vi "CfgManager Main Test Suite.vi"() -> ()   [LabVIEW 2013]
uses:
  source/Cache/ConfigManager.Cache.lvclass
  <vilib>/addons/_JKI Toolkits/Caraya/classes/Assert/Assert Equal Value and Type_Variant.vi
  <vilib>/addons/_JKI Toolkits/Caraya/classes/Assert/Assert Almost Equal_Float.vi
  source/Manager/Write.vi
  source/Manager/ConfigManager.lvclass
  <vilib>/addons/_JKI Toolkits/Caraya/classes/Test/Test.lvclass
  <vilib>/addons/_JKI Toolkits/Caraya/classes/Assert/Assert.lvclass
panel:
  out "error out":errorcluster
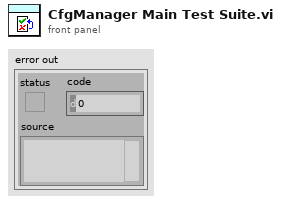
[diagram p1: front panel]
types:
  T1 = cluster{"P":dbl, "I":dbl, "D":dbl, "Type":enum16{"Manual", "Automatic"}}
  T2 = cluster{"P":dbl, "Type":enum16{"Manual", "Automatic"}}
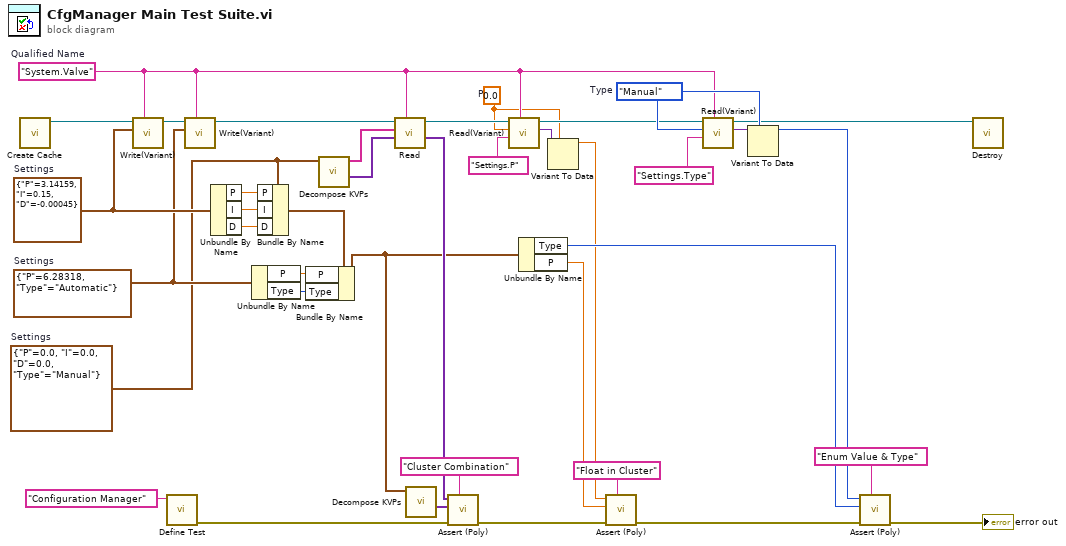
[diagram p0: block diagram]
diagram:
  w13 = 0.0  # P
  w1 = T1 {"P"=0.0, "I"=0.0, "D"=0.0, "Type"=enum."Manual"}  # Settings
  w32 = enum16{"Manual", "Automatic"}."Manual"  # Type
  w6 = T2 {"P"=6.28318, "Type"=enum."Automatic"}  # Settings
  w11 = cluster{"P":dbl, "I":dbl, "D":dbl} {"P"=3.14159, "I"=0.15, "D"=-0.00045}  # Settings
  w26 = "System.Valve"  # Qualified Name
  n1 = call "Create Cache.vi"() -> ("ConfigManager.Cache"=w39:refnum<class "ConfigManager.Cache.lvclass">)  [unwired: 11 in]
  n2 = call "Write(Variant).vi"("Qualified Name"=w26, "value"=w11, "ConfigManager in"=w39) -> ("ConfigManager out"=w35:refnum<class "ConfigManager.Cache.lvclass">)  [unwired: 6 in, 2 out]
  n3 = call <vilib>:"Define Test.vi"("Label (VI Title)"="Configuration Manager") -> ("error out"=w21:errorcluster)  [unwired: 10 in]
  n4 = call "Write(Variant).vi"("Qualified Name"=w26, "value"=w6, "ConfigManager in"=w35) -> ("ConfigManager out"=w25:refnum<class "ConfigManager.Cache.lvclass">)  [unwired: 6 in, 2 out]
  n5 = Unbundle By Name(w11) -> ("P"=w10:dbl, "I"=w9:dbl, "D"=w8:dbl)
  n6 = Unbundle By Name(w6) -> ("P"=w5:dbl, "Type"=w7:enum16{"Manual", "Automatic"})
  n7 = Bundle By Name(cluster=w1, "P"=w10, "I"=w9, "D"=w8) -> (w2:T1)
  n8 = Bundle By Name(cluster=w2, "P"=w5, "Type"=w7) -> (w4:T1)
  n9 = call "Decompose KVPs.vi"("value"=w1) -> ("Values"=w23:variant[], "Keys"=w24:string[])  [unwired: 9 in]
  n10 = call "Read.vi"("Qualified Name"=w26, "Default Values"=w23, "keys in"=w24, "ConfigManager in"=w25) -> ("Values"=w20:variant[], "ConfigManager out"=w28:refnum<class "ConfigManager.Cache.lvclass">)  [unwired: 2 in, 4 out]
  n11 = call "Decompose KVPs.vi"("value"=w4) -> ("Values"=w19:variant[])  [unwired: 9 in, 1 out]
  n12 = call-poly <vilib>:"Assert (Poly).vi"("Label"="Cluster Combination", "error in (no error)"=w21, "Y"=w19, "X"=w20) -> ("error out"=w16:errorcluster)  [unwired: 7 in]
  n13 = call "Read(Variant).vi"("Qualified Name"=w26, "Name (empty: type name)"="Settings.P", "Type"=w13, "ConfigManager in"=w28) -> ("value"=w14:variant, "ConfigManager out"=w27:refnum<class "ConfigManager.Cache.lvclass">)  [unwired: 3 in, 3 out]
  n14 = Unbundle By Name(w4) -> ("Type"=w30:enum16{"Manual", "Automatic"}, "P"=w3:dbl)
  n15 = Variant To Data(type=w13, Variant=w14) -> (data=w12:dbl)  [unwired: 1 in, 1 out]
  n16 = call-poly <vilib>:"Assert (Poly).vi"("Label"="Float in Cluster", "error in (no error)"=w16, "Y"=w3, "X"=w12) -> ("error out"=w15:errorcluster)  [unwired: 7 in]
  n17 = call "Read(Variant).vi"("Qualified Name"=w26, "Name (empty: type name)"="Settings.Type", "Type"=w32, "ConfigManager in"=w27) -> ("value"=w33:variant, "ConfigManager out"=w29:refnum<class "ConfigManager.Cache.lvclass">)  [unwired: 3 in, 3 out]
  n18 = Variant To Data(type=w32, Variant=w33) -> (data=w31:enum16{"Manual", "Automatic"})  [unwired: 1 in, 1 out]
  n19 = call-poly <vilib>:"Assert (Poly).vi"("Label"="Enum Value & Type", "error in (no error)"=w15, "Y"=w30, "X"=w31) -> ("error out"=→"error out":errorcluster)  [unwired: 7 in]
  n20 = call-dynamic "Destroy.vi"("ConfigManager.Cache in"=w29) -> ()  [unwired: 9 in, 2 out]
